vi "Helper Loop Core.vi"(8 "error in":errorcluster, 11 "Event Registration Refnum":refnum<event-registration>) -> (0 "error out":errorcluster)   [LabVIEW 2020, in "Helper Loop.lvclass"]
doc: "ヘルパーループ。周期的にメッセージとメッセージデータをエンキューします。\nEvent Resistration RefnumはStart Periodic Enqueue Message.viでこのVIを呼び出す直前に作成します\nMHLでの実際の処理時間は考慮していないため、MHLのキューが貯まらないように注意してください。"
uses:
  Helper Loop.lvclass
  Helper Loop.lvclass/Helper Loop.ctl
  support/Message Queue/Message Queue.lvlib
  support/Message Queue/Message Cluster.ctl
  <vilib>/Utility/error.llb/DialogType.ctl
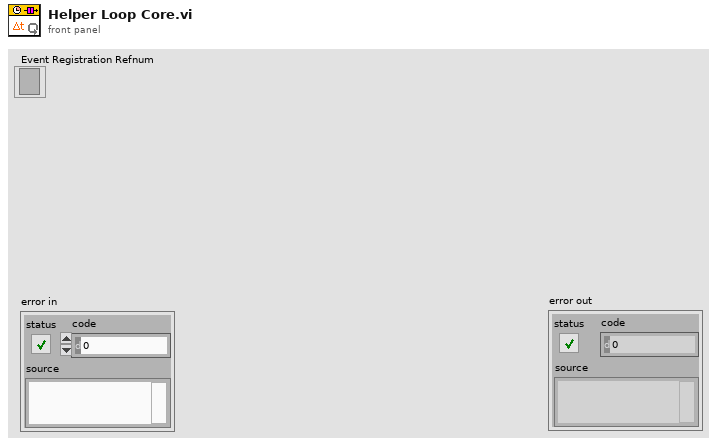
[diagram p1: front panel]
types:
  T1 = typedef "DialogType.ctl" = u16
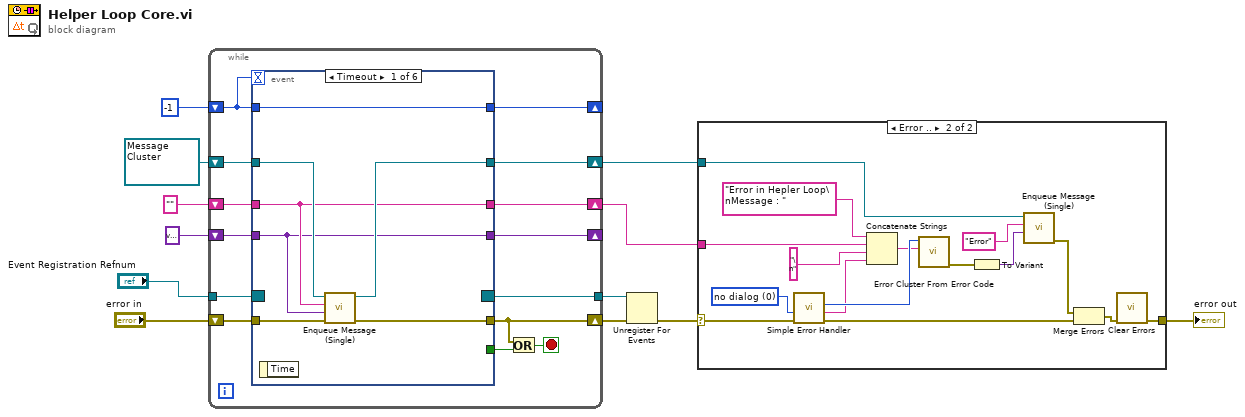
[diagram p0: block diagram]
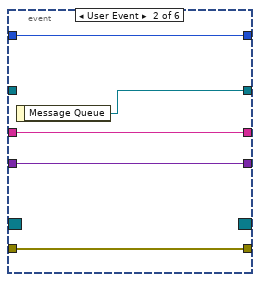
[diagram p3: hidden frame]
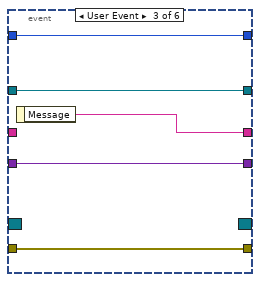
[diagram p4: hidden frame]
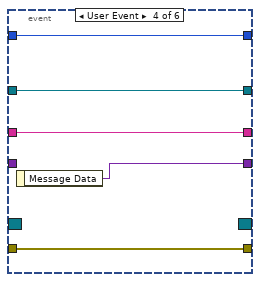
[diagram p5: hidden frame]
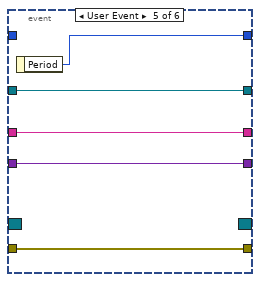
[diagram p6: hidden frame]
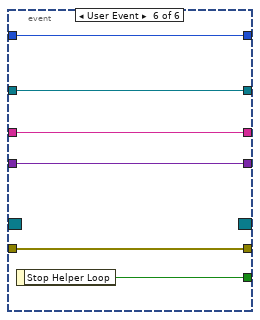
[diagram p7: hidden frame]
diagram:
  n1 = while {
    tunnel: "Event Registration Refnum" -> [w26]
    shift-right: [w14] -> w11
    shift-left: "error in" -> [w23]
    shift-right: [w25] -> _
    shift-left: -1 -> [w24]
    tunnel: [w22] -> w10
    shift-right: [w20] -> w4
    shift-left: refnum<queue> refnum ("dup Message Queue") -> [w21]
    shift-right: [w18] -> w5
    shift-left: "" -> [w19]
    shift-right: [w16] -> _
    shift-left: variant ("Message Data") -> [w17]
    stop <- w13 stop-if-true
    n2 = event shown="[0] Timeout" {
      selector: w26 -> [_ _ _ _ _ _]
      dyn-events: [_ _ _ _ _ _] -> w22
      timeout: w24 -> [_ _ _ _ _ _]
      tunnel: [w33 w34 w42 w48 w49 w59] -> w25
      tunnel: w24 -> [w33 w34 w42 w48 _ w59]
      tunnel: w23 -> [w32 w38 w39 w47 w53 w58]
      tunnel: [w31 w38 w39 w47 w53 w58] -> w14
      tunnel: [_ _ _ _ _ w54] -> w15
      tunnel: w21 -> [w30 _ w43 w46 w52 w57]
      tunnel: [w29 w35 w43 w46 w52 w57] -> w20
      tunnel: w19 -> [w28 w36 _ w45 w51 w56]
      tunnel: [w28 w36 w41 w45 w51 w56] -> w18
      tunnel: w17 -> [w27 w37 w40 _ w50 w55]
      tunnel: [w27 w37 w40 w44 w50 w55] -> w16
      event Timeout {
        n3 = event-data() -> ()  [unwired: 1 in, 1 out]
        n4 = call "Enqueue Message (Single).vi"("error in (no error)"=w32, "Message Data"=w27, "Message"=w28, "Message Queue"=w30) -> ("error out"=w31:errorcluster, "dup Message Queue"=w29:refnum<queue>)  [unwired: 6 in]
      }
      event User Event {
        n5 = event-data() -> ("Message Queue"=w35:refnum<queue>)  [unwired: 1 in]
      }
      event User Event {
        n6 = event-data() -> ("Message"=w41:string)  [unwired: 1 in]
      }
      event User Event {
        n7 = event-data() -> ("Message Data"=w44:variant)  [unwired: 1 in]
      }
      event User Event {
        n8 = event-data() -> ("Period"=w49:i32)  [unwired: 1 in]
      }
      event User Event {
        n9 = event-data() -> ("Stop Helper Loop"=w54:bool)  [unwired: 1 in]
      }
    }
    n10 = Or(x=w14, y=w15) -> (x .or. y?=w13:bool)
  }
  n11 = Unregister For Events(event registration refnum=w10, error in=w11) -> (error out=w6:errorcluster)
  n12 = case shown="Error .." w6 {
    selector: w6 -> [w60 w63]
    tunnel: [w60 w72] -> w3
    tunnel: w4 -> [_ w76]
    tunnel: w5 -> [_ w68]
    frame No Error {
    }
    frame Error {
      w73 = T1 0 items=["no dialog", "OK message", "continue or stop message", "OK message + warnings", "continue/stop + warnings"] ("type of dialog (OK msg:1)")
      n13 = call <vilib>:"Simple Error Handler.vi"("type of dialog (OK msg:1)"=w73, "error in (no error)"=w63) -> ("code out"=w70:i32, "source out"=w67:string, "error out"=w61:errorcluster)  [unwired: 3 in, 2 out]
      n14 = Concatenate Strings("Error in Hepler Loop\nMessage : " ("string"), w68, "\n" ("string"), w67) -> (w65:string)
      n15 = call <vilib>:"Error Cluster From Error Code.vi"("error message (\"\")"=w65, "error code (0)"=w70) -> ("error out"=w71:errorcluster)  [unwired: 7 in]
      n16 = To Variant(anything=w71) -> (Variant=w75:variant)
      n17 = call "Enqueue Message (Single).vi"("Message Data"=w75, "Message"="Error", "Message Queue"=w76) -> ("error out"=w64:errorcluster)  [unwired: 7 in, 1 out]
      n18 = Merge Errors(w64, w61) -> (w62:errorcluster)
      n19 = call <vilib>:"Clear Errors.vi"("error in (no error)"=w62) -> ("error out"=w72:errorcluster)  [unwired: 5 in, 1 out]
    }
  }
  "error out" <- w3
